vi "ReadFile.vi"(8 "error in (no error)":errorcluster, 11 "object in":refnum<class "ChannelsManager.lvclass">) -> (0 "error out":errorcluster, 3 "object out":refnum<class "ChannelsManager.lvclass">)   [LabVIEW 2021, in "Channel.lvlib" / "ChannelsManager.lvlib" / "ChannelsManager.lvclass"]
doc: "Reads the channels File"
uses:
  ChannelsManager.lvclass
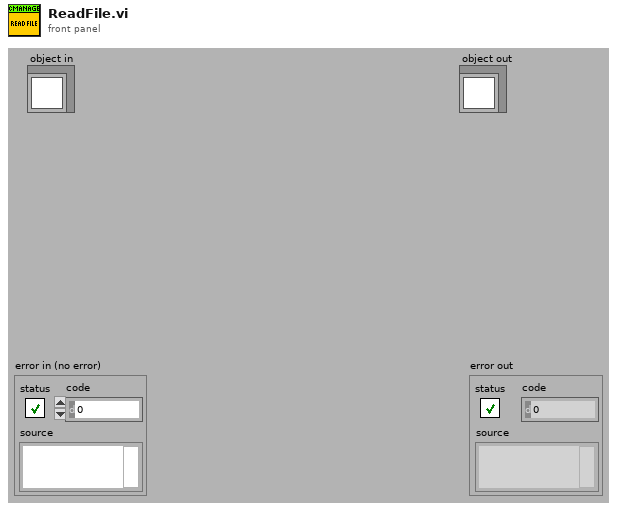
[diagram p1: front panel]
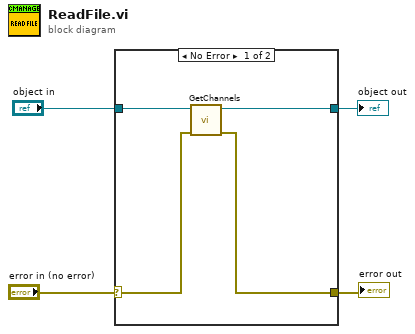
[diagram p0: block diagram]
diagram:
  n1 = case shown="No Error" "error in (no error)" {
    selector: "error in (no error)" -> [w7 w10]
    tunnel: [w6 w10] -> w3
    tunnel: [w5 w9] -> w1
    tunnel: "object in" -> [w8 w9]
    frame No Error {
      n2 = call-dynamic "GetChannels.vi"("error in (no error)"=w7, "object in"=w8) -> ("error out"=w6:errorcluster, "object out"=w5:refnum<class "ChannelsManager.lvclass">)  [unwired: 7 in, 1 out]
    }
    frame Error {
    }
  }
  "error out" <- w3
  "object out" <- w1
